vi "Create.vi"(7 "Size":i32, 8 "error in (no error)":errorcluster, 10 "Channel Info":T1) -> (0 "error out":errorcluster, 3 "Channel Buffer DBL out":refnum<class "Channel Buffer DBL.lvclass">)   [LabVIEW 2020, in "VolatusHistorian.lvlib" / "Channel Buffer DBL.lvclass"]
uses:
  Channel Buffer DBL.lvclass
  lv-vecto/Vecto/Channel Info.ctl
  Channel Buffer DBL.lvclass/Channel Buffer DBL.ctl
  lv-vecto/VectoConfig/VectoConfig.lvlib
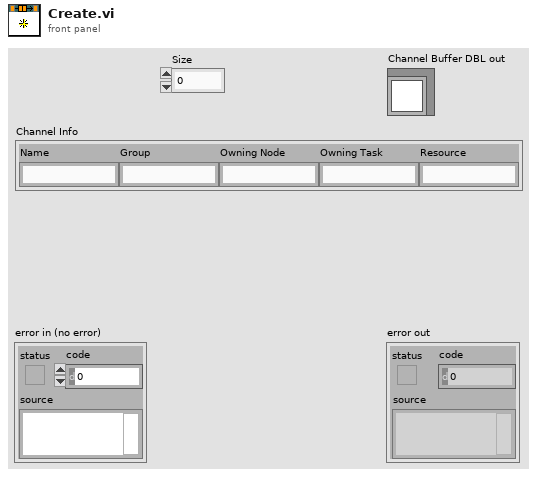
[diagram p1: front panel]
types:
  T1 = typedef "VectoConfig.lvlib/Channel Info.ctl" = cluster{"Name":string, "Group":string, "Owning Node":string, "Owning Task":string, "Resource":string}
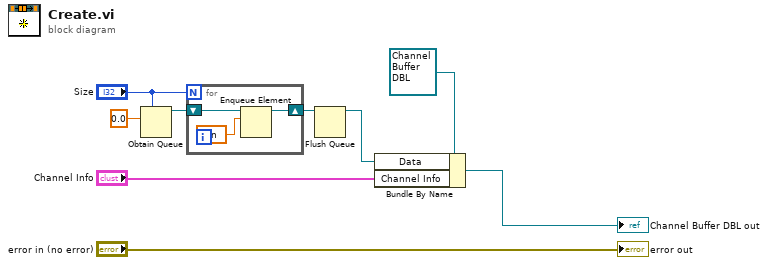
[diagram p0: block diagram]
diagram:
  n1 = Obtain Queue(max queue size (-1, unlimited)="Size", element data type=0.0) -> (queue out=w3:refnum<queue>)  [unwired: 3 in, 2 out]
  n2 = for {
    N: "Size" -> [_]
    shift-right: [w10] -> w2
    shift-left: w3 -> [w12]
    n3 = Enqueue Element(queue=w12, element=nan) -> (queue out=w10:refnum<queue>)  [unwired: 2 in, 2 out]
  }
  n4 = Flush Queue(queue=w2) -> (queue out=w1:refnum<queue>)  [unwired: 1 in, 2 out]
  n5 = Bundle By Name(cluster=refnum<class "Channel Buffer DBL.lvclass"> refnum ("Channel Buffer DBL in"), "Data"=w1, "Channel Info"="Channel Info") -> (→"Channel Buffer DBL out":refnum<class "Channel Buffer DBL.lvclass">)
  "error out" <- "error in (no error)"
